vi "Read Weiss File.vi"(11 "Path":path=path "D:/同步空间/曲线生成/原始曲线/1-1、伟思1 原始数据 --mande.x66") -> (3 "Data Series":T1[](array[typedef]))   [LabVIEW 2020, in "Data Viewer.lvlib"]
uses:
  Data Viewer.lvlib
  Data Serie--cluster.ctl
  File Type--enum.ctl
  <vilib>/Utility/file.llb/Read Delimited Spreadsheet (string).vi
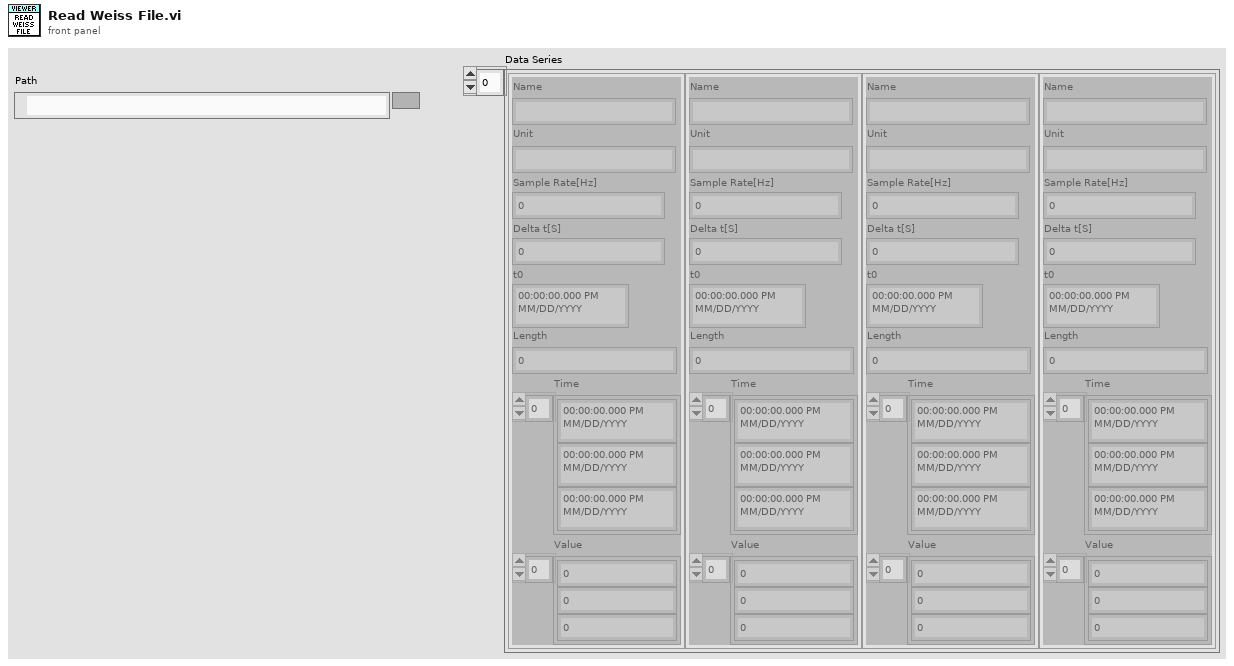
[diagram p1: front panel]
types:
  T1 = typedef "Data Viewer.lvlib/Data Serie--cluster.ctl" = cluster{"Name":string, "Unit":string, "Sample Rate[Hz]":dbl, "Delta t[S]":dbl, "t0":timestamp, "Length":i32, "Time":timestamp[], "Value":dbl[]}
  T2 = typedef "Data Viewer.lvlib/File Type--enum.ctl" = enum16{"伟思环境箱", "增达环境箱", "广五所环境箱", "无纸记录仪", "帕捷SA00339", "记录仪840", "记录仪8400", "记录仪MR888", "*.csv"}
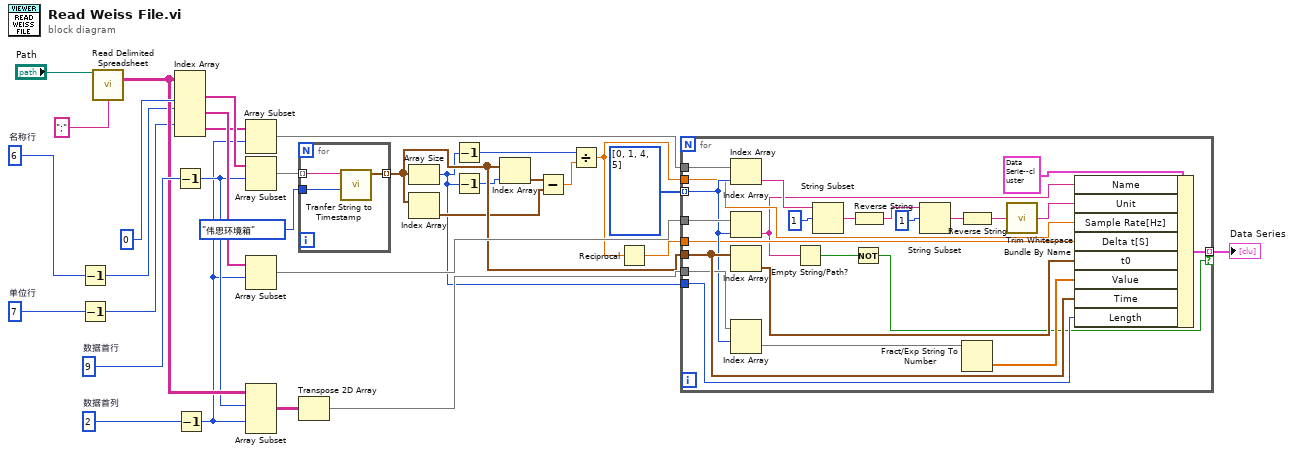
[diagram p0: block diagram]
diagram:
  w23 = 2  # 数据首列
  w24 = 9  # 数据首行
  w26 = 7  # 单位行
  w28 = 6  # 名称行
  n1 = Decrement(x=w28) -> (x-1=w6:i32)
  n2 = Decrement(x=w26) -> (x-1=w5:i32)
  n3 = call-poly <vilib>:"Read Delimited Spreadsheet.vi"("file path (dialog if empty)"="Path", "delimiter (\\t)"=";" ("delimiter (\\t)")) -> ("all rows"=w7:string[][])  [unwired: 8 in, 5 out]
  n4 = Index Array(array=w7, index (col) #1=0 ("disabled index (col)"), index (row) #2=w6, index (row) #3=w5) -> (element #1=w31:string[], element #2=w27:string[], element #3=w25:string[])  [unwired: 3 in]
  n5 = Decrement(x=w24) -> (x-1=w4:i32)
  n6 = Decrement(x=w23) -> (x-1=w3:i32)
  n7 = Array Subset(array=w25, index=w3) -> (w19:string[])  [unwired: 1 in]
  n8 = Array Subset(array=w31, index=w4) -> (w30:string[])  [unwired: 1 in]
  n9 = Array Subset(array=w27, index=w3) -> (w20:string[])  [unwired: 1 in]
  n10 = Array Subset(array=w7, index (row)=w4, index (col)=w3) -> (w22:string[][])  [unwired: 2 in]
  n11 = for {
    tunnel: w30 -> [w35] mode=indexing
    tunnel: File_Type--enum."伟思环境箱" ("File Type") -> [w34]
    tunnel: [w33] -> w17 mode=indexing
    n12 = call "Tranfer String to Timestamp.vi"("File Type"=w34, "String"=w35) -> ("time stamp"=w33:timestamp)  [unwired: 9 in]
  }
  n13 = Transpose 2D Array(2D array=w22) -> (transposed array=w18:string[][])
  n14 = Array Size(array=w17) -> (size(s)=w1:i32)
  n15 = Index Array(array=w17) -> (element=w14:timestamp)  [unwired: 1 in]
  n16 = Decrement(x=w1) -> (x-1=w2:i32)
  n17 = Decrement(x=w1) -> (x-1=w16:i32)
  n18 = Index Array(array=w17, index=w16) -> (element=w15:timestamp)
  n19 = Subtract(x=w15, y=w14) -> (x-y=w13:dbl)
  n20 = Divide(x=w2, y=w13) -> (x/y=w12:dbl)
  n21 = Reciprocal(x=w12) -> (1/x=w11:dbl)
  n22 = for {
    tunnel: i32[] [0, 1, 4, 5] -> [w53] mode=indexing
    tunnel: w20 -> [w58]
    tunnel: w19 -> [w57]
    tunnel: w18 -> [w54]
    tunnel: w17 -> [w55]
    tunnel: w12 -> [w50]
    tunnel: w11 -> [w49]
    tunnel: [w48] -> w10 mode=indexing if=w37
    tunnel: w1 -> [w39]
    n23 = Index Array(array=w57, index=w53) -> (element=w47:string)
    n24 = Index Array(array=w58, index=w53) -> (element=w36:string)
    n25 = Index Array(array=w55) -> (element=w56:timestamp)  [unwired: 1 in]
    n26 = Index Array(array=w54, index (row)=w53) -> (element=w52:string[])  [unwired: 1 in]
    n27 = Empty String/Path?(string/path=w36) -> (empty?=w38:bool)
    n28 = String Subset(string=w47, offset (0)=1) -> (substring=w45:string)  [unwired: 1 in]
    n29 = Not(x=w38) -> (.not. x?=w37:bool)
    n30 = Reverse String(1:w45) -> (0:w42:string)
    n31 = String Subset(string=w42, offset (0)=1) -> (substring=w44:string)  [unwired: 1 in]
    n32 = Reverse String(1:w44) -> (0:w41:string)
    n33 = Fract/Exp String To Number(string=w52) -> (number=w51:dbl[])  [unwired: 3 in, 1 out]
    n34 = call <vilib>:"Trim Whitespace.vi"("string"=w41) -> ("trimmed string"=w40:string)  [unwired: 1 in]
    n35 = Bundle By Name(cluster=T1 {"Name"="", "Unit"="", "Sample Rate[Hz]"=0.0, "Delta t[S]"=0.0, "t0"=timestamp(0 s since 1904-01-01), "Length"=0, "Time"=[], "Value"=[]} ("Data Serie"), "Name"=w36, "Unit"=w40, "Sample Rate[Hz]"=w50, "Delta t[S]"=w49, "t0"=w56, "Value"=w51, "Time"=w55, "Length"=w39) -> (w48:T1)
  }
  "Data Series" <- w10
